vi "OFDM_SuperpositionedBitDetectV3.vi"(5 "Alpha":dbl, 6 "Input symbolsLP":cdb[](array[numeric]) format="%.2f", 7 "Input symbolsHP":cdb[](array[numeric]) format="%.2f", 8 "error in (no error)":errorcluster, 9 "Modulation type LP":enum16{"QPSK(4QAM)", "64QAM", "16QAM", "BPSK"}(ring), 10 "Modulation type":enum16{"QPSK(4QAM)", "64QAM", "16QAM", "BPSK"}(ring), 11 "Input symbols":cdb[](array[numeric]) format="%.2f") -> (0 "error out":errorcluster, 1 "OutputbitsHP":i8[](array[numeric]) caption="Output bits", 2 "SNR dB HP":dbl, 3 "OutputbitsLP":i8[](array[numeric]) caption="Output bits", 4 "SNR dB LP":dbl)   [LabVIEW 2022 SP3]
uses:
  <vilib>/addons/Modulation/Digital/General/MT Map QAM Symbols to Bits.vi
  <vilib>/addons/Modulation/Digital/General/MT Map Bits to QAM Symbols.vi
  <vilib>/addons/Modulation/Digital/General/MT Map PSK Symbols to Bits.vi
  <vilib>/addons/Modulation/Digital/General/MT Map Bits to PSK Symbols.vi
  <vilib>/addons/Modulation/niDMT.lvlib
panel:
  out "x-y":cdb[](array[numeric])
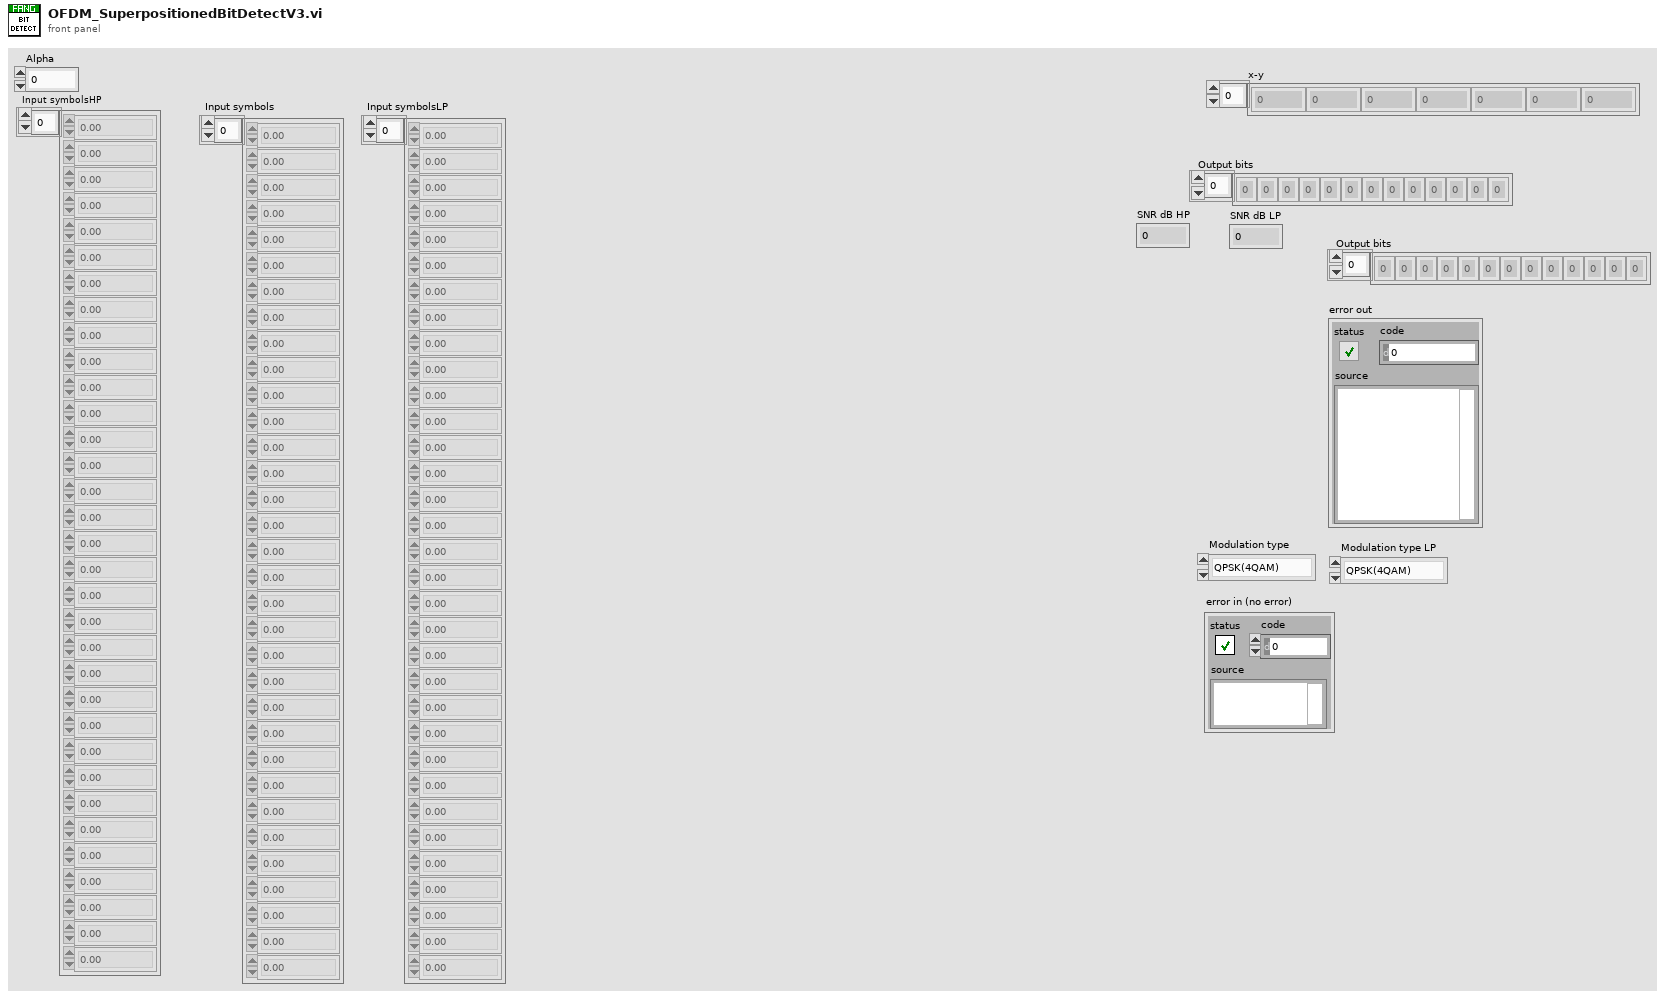
[diagram p1: front panel]
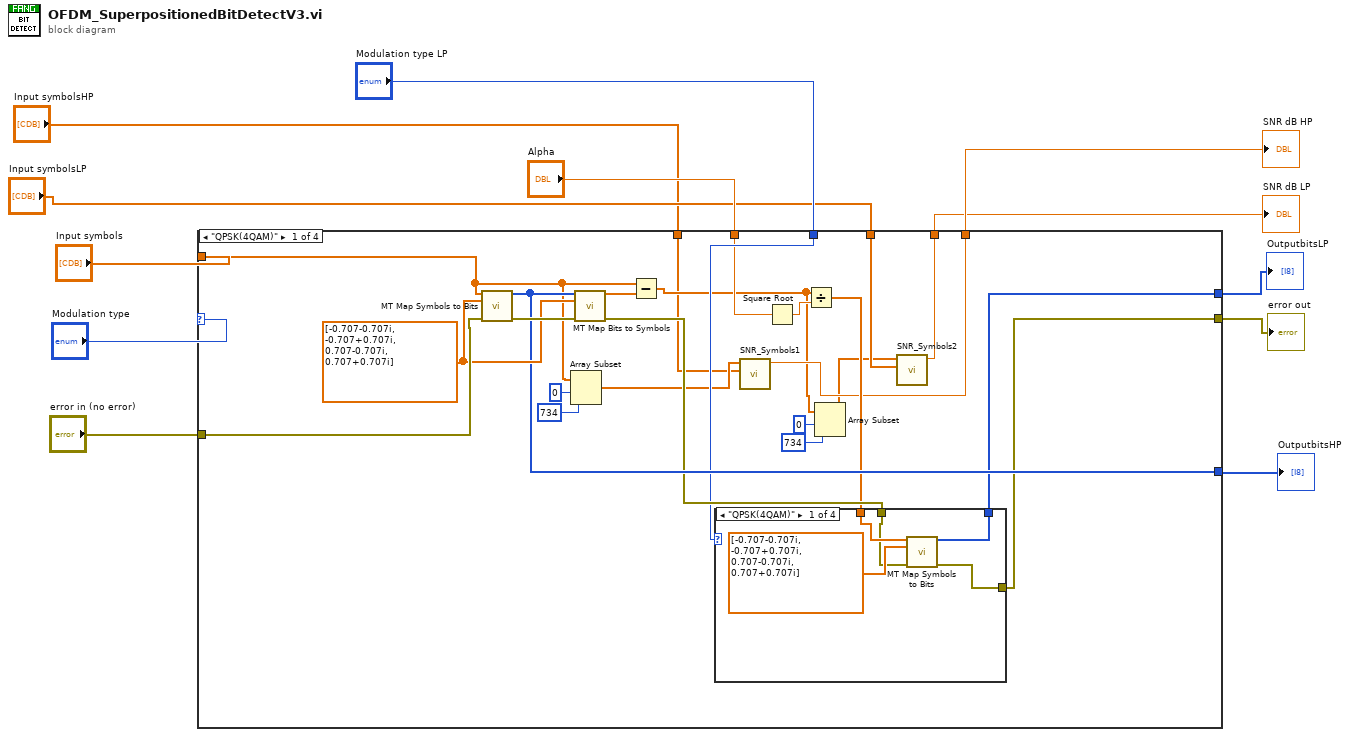
[diagram p0: block diagram]
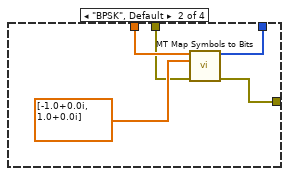
[diagram p2: hidden frame]
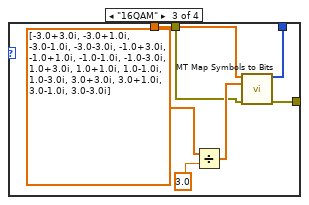
[diagram p3: hidden frame]
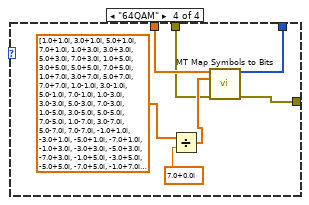
[diagram p4: hidden frame]
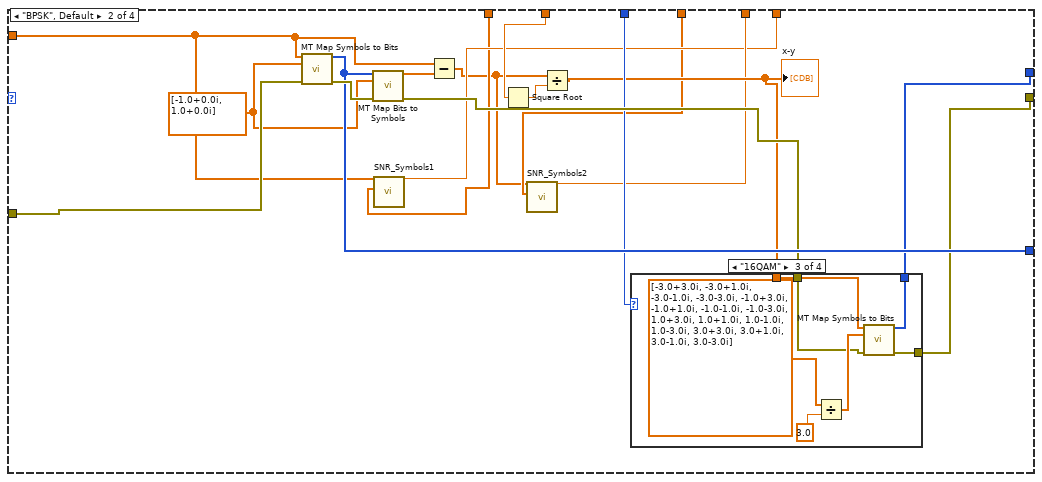
[diagram p5: hidden frame]
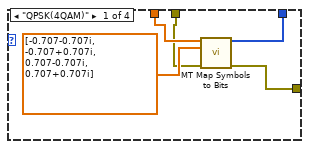
[diagram p6: hidden frame]
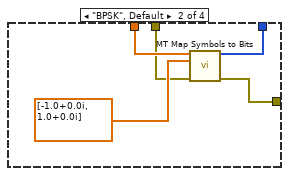
[diagram p7: hidden frame]
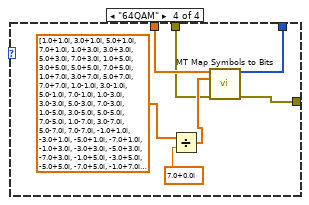
[diagram p8: hidden frame]
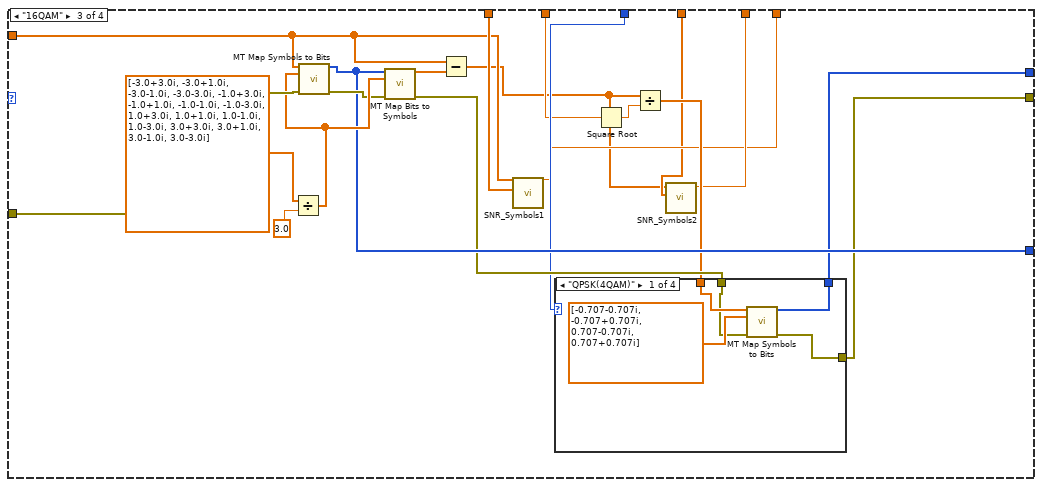
[diagram p9: hidden frame]
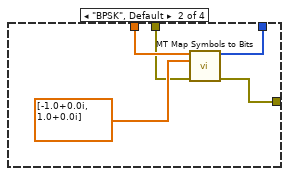
[diagram p10: hidden frame]
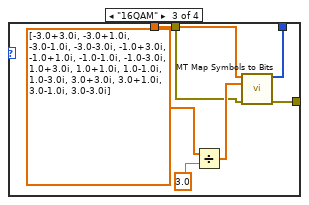
[diagram p11: hidden frame]
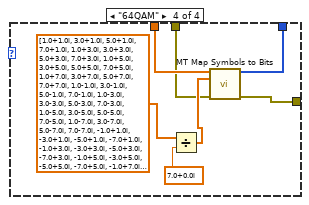
[diagram p12: hidden frame]
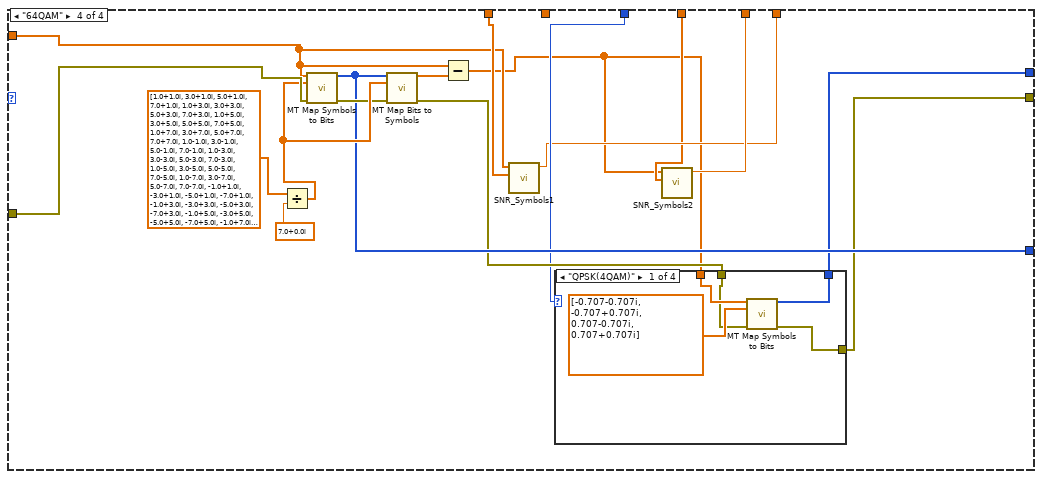
[diagram p13: hidden frame]
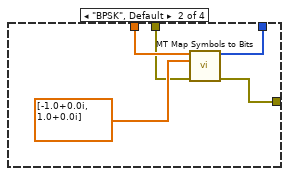
[diagram p14: hidden frame]
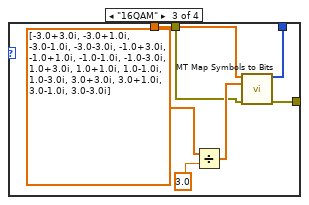
[diagram p15: hidden frame]
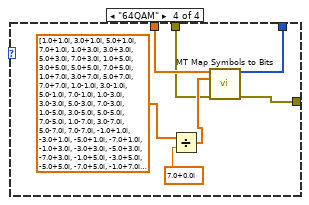
[diagram p16: hidden frame]
diagram:
  n1 = case shown="\"QPSK(4QAM)\"" "Modulation type" {
    tunnel: "Input symbols" -> [w14 w62 w104 w148]
    tunnel: "error in (no error)" -> [w36 w78 w122 w161]
    tunnel: [w30 w73 w113 w154] -> w9
    tunnel: [w31 w72 w114 w155] -> w8
    tunnel: [w33 w75 w116 w157] -> w7
    tunnel: "Modulation type LP" -> [w29 w70 w112 w153]
    tunnel: "Alpha" -> [w26 w67 w109 _]
    tunnel: "Input symbolsHP" -> [w15 w64 w106 w150]
    tunnel: "Input symbolsLP" -> [w25 w63 w105 w149]
    tunnel: [w24 w65 w107 w151] -> w3
    tunnel: [w23 w66 w108 w152] -> w2
    frame "QPSK(4QAM)" {
      w34 = cdb[] [-0.707-0.707i, -0.707+0.707i, 0.707-0.707i, 0.707+0.707i] ("symbol map")
      n2 = call-poly <vilib>:"MT Map Symbols to Bits.vi"("symbols"=w14, "symbol map"=w34, "error in (no error)"=w36) -> ("output bit stream"=w33:i8[], "error out"=w35:errorcluster)  [unwired: 11 in]
      n3 = Array Subset(array=w14, index=0, length=734) -> (w22:cdb[])
      n4 = call-poly <vilib>:"MT Map Bits to Symbols.vi"("input bit stream"=w33, "symbol map"=w34, "error in (no error)"=w35) -> ("symbols"=w13:cdb[], "error out"=w32:errorcluster)  [unwired: 11 in]
      n5 = Subtract(x=w14, y=w13) -> (x-y=w16:cdb[])
      n6 = call "SNR_Symbols1.vi"("Ideal Symbols"=w15, "Received symbols"=w22) -> ("SNR dB"=w24:dbl)  [unwired: 9 in]
      n7 = Square Root(x=w26) -> (sqrt(x)=w28:dbl)
      n8 = Divide(x=w16, y=w28) -> (x/y=w27:cdb[])
      n9 = case shown="\"QPSK(4QAM)\"" w29 {
        tunnel: w27 -> [w40 w45 w50 w57]
        tunnel: [w38 w44 w49 w55] -> w30
        tunnel: [w37 w42 w48 w54] -> w31
        tunnel: w32 -> [w39 w43 w47 w56]
        frame "QPSK(4QAM)" {
          n10 = call-poly <vilib>:"MT Map Symbols to Bits.vi"("symbols"=w40, "symbol map"=cdb[] [-0.707-0.707i, -0.707+0.707i, 0.707-0.707i, 0.707+0.707i], "error in (no error)"=w39) -> ("output bit stream"=w38:i8[], "error out"=w37:errorcluster)  [unwired: 11 in]
        }
        frame "BPSK", Default {
          n11 = call-poly <vilib>:"MT Map Symbols to Bits.vi"("symbols"=w45, "symbol map"=cdb[] [-1.0+0.0i, 1.0+0.0i], "error in (no error)"=w43) -> ("output bit stream"=w44:i8[], "error out"=w42:errorcluster)  [unwired: 11 in]
        }
        frame "16QAM" {
          n12 = Divide(x=cdb[] [-3.0+3.0i, -3.0+1.0i, -3.0-1.0i, -3.0-3.0i, -1.0+3.0i, -1.0+1.0i, -1.0-1.0i, -1.0-3.0i, 1.0+3.0i, 1.0+1.0i, 1.0-1.0i, 1.0-3.0i, 3.0+3.0i, 3.0+1.0i, 3.0-1.0i, 3.0-3.0i] ("symbol map"), y=3.0) -> (x/y=w51:cdb[])
          n13 = call-poly <vilib>:"MT Map Symbols to Bits.vi"("symbols"=w50, "symbol map"=w51, "error in (no error)"=w47) -> ("output bit stream"=w49:i8[], "error out"=w48:errorcluster)  [unwired: 11 in]
        }
        frame "64QAM" {
          n14 = Divide(x=cdb[] [1.0+1.0i, 3.0+1.0i, 5.0+1.0i, 7.0+1.0i, 1.0+3.0i, 3.0+3.0i, 5.0+3.0i, 7.0+3.0i, 1.0+5.0i, 3.0+5.0i, 5.0+5.0i, 7.0+5.0i, 1.0+7.0i, 3.0+7.0i, 5.0+7.0i, 7.0+7.0i, 1.0-1.0i, 3.0-1.0i, 5.0-1.0i, 7.0-1.0i, 1.0-3.0i, 3.0-3.0i, 5.0-3.0i, 7.0-3.0i, 1.0-5.0i, 3.0-5.0i, 5.0-5.0i, 7.0-5.0i, 1.0-7.0i, 3.0-7.0i, 5.0-7.0i, 7.0-7.0i, -1.0+1.0i, -3.0+1.0i, -5.0+1.0i, -7.0+1.0i, -1.0+3.0i, -3.0+3.0i, -5.0+3.0i, -7.0+3.0i, -1.0+5.0i, -3.0+5.0i, -5.0+5.0i, -7.0+5.0i, -1.0+7.0i, -3.0+7.0i, -5.0+7.0i, -7.0+7.0i, -1.0-1.0i, -3.0-1.0i, -5.0-1.0i, -7.0-1.0i, -1.0-3.0i, -3.0-3.0i, -5.0-3.0i, -7.0-3.0i, -1.0-5.0i, -3.0-5.0i, -5.0-5.0i, -7.0-5.0i, -1.0-7.0i, -3.0-7.0i, -5.0-7.0i, -7.0-7.0i] ("appended array"), y=cdb 7.0+0.0i) -> (x/y=w58:cdb[])
          n15 = call-poly <vilib>:"MT Map Symbols to Bits.vi"("symbols"=w57, "symbol map"=w58, "error in (no error)"=w56) -> ("output bit stream"=w55:i8[], "error out"=w54:errorcluster)  [unwired: 11 in]
        }
      }
      n16 = Array Subset(array=w16, index=0, length=734) -> (w17:cdb[])
      n17 = call "SNR_Symbols2.vi"("Ideal Symbols"=w25, "Received symbols"=w17) -> ("SNR dB"=w23:dbl)  [unwired: 9 in]
    }
    frame "BPSK", Default {
      w74 = cdb[] [-1.0+0.0i, 1.0+0.0i] ("symbol map")
      n18 = call-poly <vilib>:"MT Map Symbols to Bits.vi"("symbols"=w62, "symbol map"=w74, "error in (no error)"=w78) -> ("output bit stream"=w75:i8[], "error out"=w77:errorcluster)  [unwired: 11 in]
      n19 = call-poly <vilib>:"MT Map Bits to Symbols.vi"("input bit stream"=w75, "symbol map"=w74, "error in (no error)"=w77) -> ("symbols"=w76:cdb[], "error out"=w71:errorcluster)  [unwired: 11 in]
      n20 = call "SNR_Symbols1.vi"("Ideal Symbols"=w64, "Received symbols"=w62) -> ("SNR dB"=w65:dbl)  [unwired: 9 in]
      n21 = Subtract(x=w62, y=w76) -> (x-y=w61:cdb[])
      n22 = Square Root(x=w67) -> (sqrt(x)=w68:dbl)
      n23 = call "SNR_Symbols2.vi"("Ideal Symbols"=w63, "Received symbols"=w61) -> ("SNR dB"=w66:dbl)  [unwired: 9 in]
      n24 = Divide(x=w61, y=w68) -> (x/y=w69:cdb[])
      "x-y" <- w69
      n25 = case shown="\"16QAM\"" w70 {
        tunnel: w69 -> [w82 w87 w92 w99]
        tunnel: [w80 w86 w91 w97] -> w73
        tunnel: [w79 w84 w90 w96] -> w72
        tunnel: w71 -> [w81 w85 w89 w98]
        frame "QPSK(4QAM)" {
          n26 = call-poly <vilib>:"MT Map Symbols to Bits.vi"("symbols"=w82, "symbol map"=cdb[] [-0.707-0.707i, -0.707+0.707i, 0.707-0.707i, 0.707+0.707i], "error in (no error)"=w81) -> ("output bit stream"=w80:i8[], "error out"=w79:errorcluster)  [unwired: 11 in]
        }
        frame "BPSK", Default {
          n27 = call-poly <vilib>:"MT Map Symbols to Bits.vi"("symbols"=w87, "symbol map"=cdb[] [-1.0+0.0i, 1.0+0.0i], "error in (no error)"=w85) -> ("output bit stream"=w86:i8[], "error out"=w84:errorcluster)  [unwired: 11 in]
        }
        frame "16QAM" {
          n28 = Divide(x=cdb[] [-3.0+3.0i, -3.0+1.0i, -3.0-1.0i, -3.0-3.0i, -1.0+3.0i, -1.0+1.0i, -1.0-1.0i, -1.0-3.0i, 1.0+3.0i, 1.0+1.0i, 1.0-1.0i, 1.0-3.0i, 3.0+3.0i, 3.0+1.0i, 3.0-1.0i, 3.0-3.0i] ("symbol map"), y=3.0) -> (x/y=w93:cdb[])
          n29 = call-poly <vilib>:"MT Map Symbols to Bits.vi"("symbols"=w92, "symbol map"=w93, "error in (no error)"=w89) -> ("output bit stream"=w91:i8[], "error out"=w90:errorcluster)  [unwired: 11 in]
        }
        frame "64QAM" {
          n30 = Divide(x=cdb[] [1.0+1.0i, 3.0+1.0i, 5.0+1.0i, 7.0+1.0i, 1.0+3.0i, 3.0+3.0i, 5.0+3.0i, 7.0+3.0i, 1.0+5.0i, 3.0+5.0i, 5.0+5.0i, 7.0+5.0i, 1.0+7.0i, 3.0+7.0i, 5.0+7.0i, 7.0+7.0i, 1.0-1.0i, 3.0-1.0i, 5.0-1.0i, 7.0-1.0i, 1.0-3.0i, 3.0-3.0i, 5.0-3.0i, 7.0-3.0i, 1.0-5.0i, 3.0-5.0i, 5.0-5.0i, 7.0-5.0i, 1.0-7.0i, 3.0-7.0i, 5.0-7.0i, 7.0-7.0i, -1.0+1.0i, -3.0+1.0i, -5.0+1.0i, -7.0+1.0i, -1.0+3.0i, -3.0+3.0i, -5.0+3.0i, -7.0+3.0i, -1.0+5.0i, -3.0+5.0i, -5.0+5.0i, -7.0+5.0i, -1.0+7.0i, -3.0+7.0i, -5.0+7.0i, -7.0+7.0i, -1.0-1.0i, -3.0-1.0i, -5.0-1.0i, -7.0-1.0i, -1.0-3.0i, -3.0-3.0i, -5.0-3.0i, -7.0-3.0i, -1.0-5.0i, -3.0-5.0i, -5.0-5.0i, -7.0-5.0i, -1.0-7.0i, -3.0-7.0i, -5.0-7.0i, -7.0-7.0i] ("appended array"), y=cdb 7.0+0.0i) -> (x/y=w100:cdb[])
          n31 = call-poly <vilib>:"MT Map Symbols to Bits.vi"("symbols"=w99, "symbol map"=w100, "error in (no error)"=w98) -> ("output bit stream"=w97:i8[], "error out"=w96:errorcluster)  [unwired: 11 in]
        }
      }
    }
    frame "16QAM" {
      n32 = Divide(x=cdb[] [-3.0+3.0i, -3.0+1.0i, -3.0-1.0i, -3.0-3.0i, -1.0+3.0i, -1.0+1.0i, -1.0-1.0i, -1.0-3.0i, 1.0+3.0i, 1.0+1.0i, 1.0-1.0i, 1.0-3.0i, 3.0+3.0i, 3.0+1.0i, 3.0-1.0i, 3.0-3.0i] ("symbol map"), y=3.0) -> (x/y=w119:cdb[])
      n33 = call-poly <vilib>:"MT Map Symbols to Bits.vi"("symbols"=w104, "symbol map"=w119, "error in (no error)"=w122) -> ("output bit stream"=w116:i8[], "error out"=w117:errorcluster)  [unwired: 11 in]
      n34 = call-poly <vilib>:"MT Map Bits to Symbols.vi"("input bit stream"=w116, "symbol map"=w119, "error in (no error)"=w117) -> ("symbols"=w118:cdb[], "error out"=w115:errorcluster)  [unwired: 11 in]
      n35 = Subtract(x=w104, y=w118) -> (x-y=w103:cdb[])
      n36 = call "SNR_Symbols1.vi"("Ideal Symbols"=w106, "Received symbols"=w104) -> ("SNR dB"=w107:dbl)  [unwired: 9 in]
      n37 = Square Root(x=w109) -> (sqrt(x)=w111:dbl)
      n38 = Divide(x=w103, y=w111) -> (x/y=w110:cdb[])
      n39 = case shown="\"QPSK(4QAM)\"" w112 {
        tunnel: w110 -> [w126 w131 w136 w143]
        tunnel: [w124 w130 w135 w141] -> w113
        tunnel: [w123 w128 w134 w140] -> w114
        tunnel: w115 -> [w125 w129 w133 w142]
        frame "QPSK(4QAM)" {
          n40 = call-poly <vilib>:"MT Map Symbols to Bits.vi"("symbols"=w126, "symbol map"=cdb[] [-0.707-0.707i, -0.707+0.707i, 0.707-0.707i, 0.707+0.707i], "error in (no error)"=w125) -> ("output bit stream"=w124:i8[], "error out"=w123:errorcluster)  [unwired: 11 in]
        }
        frame "BPSK", Default {
          n41 = call-poly <vilib>:"MT Map Symbols to Bits.vi"("symbols"=w131, "symbol map"=cdb[] [-1.0+0.0i, 1.0+0.0i], "error in (no error)"=w129) -> ("output bit stream"=w130:i8[], "error out"=w128:errorcluster)  [unwired: 11 in]
        }
        frame "16QAM" {
          n42 = Divide(x=cdb[] [-3.0+3.0i, -3.0+1.0i, -3.0-1.0i, -3.0-3.0i, -1.0+3.0i, -1.0+1.0i, -1.0-1.0i, -1.0-3.0i, 1.0+3.0i, 1.0+1.0i, 1.0-1.0i, 1.0-3.0i, 3.0+3.0i, 3.0+1.0i, 3.0-1.0i, 3.0-3.0i] ("symbol map"), y=3.0) -> (x/y=w137:cdb[])
          n43 = call-poly <vilib>:"MT Map Symbols to Bits.vi"("symbols"=w136, "symbol map"=w137, "error in (no error)"=w133) -> ("output bit stream"=w135:i8[], "error out"=w134:errorcluster)  [unwired: 11 in]
        }
        frame "64QAM" {
          n44 = Divide(x=cdb[] [1.0+1.0i, 3.0+1.0i, 5.0+1.0i, 7.0+1.0i, 1.0+3.0i, 3.0+3.0i, 5.0+3.0i, 7.0+3.0i, 1.0+5.0i, 3.0+5.0i, 5.0+5.0i, 7.0+5.0i, 1.0+7.0i, 3.0+7.0i, 5.0+7.0i, 7.0+7.0i, 1.0-1.0i, 3.0-1.0i, 5.0-1.0i, 7.0-1.0i, 1.0-3.0i, 3.0-3.0i, 5.0-3.0i, 7.0-3.0i, 1.0-5.0i, 3.0-5.0i, 5.0-5.0i, 7.0-5.0i, 1.0-7.0i, 3.0-7.0i, 5.0-7.0i, 7.0-7.0i, -1.0+1.0i, -3.0+1.0i, -5.0+1.0i, -7.0+1.0i, -1.0+3.0i, -3.0+3.0i, -5.0+3.0i, -7.0+3.0i, -1.0+5.0i, -3.0+5.0i, -5.0+5.0i, -7.0+5.0i, -1.0+7.0i, -3.0+7.0i, -5.0+7.0i, -7.0+7.0i, -1.0-1.0i, -3.0-1.0i, -5.0-1.0i, -7.0-1.0i, -1.0-3.0i, -3.0-3.0i, -5.0-3.0i, -7.0-3.0i, -1.0-5.0i, -3.0-5.0i, -5.0-5.0i, -7.0-5.0i, -1.0-7.0i, -3.0-7.0i, -5.0-7.0i, -7.0-7.0i] ("appended array"), y=cdb 7.0+0.0i) -> (x/y=w144:cdb[])
          n45 = call-poly <vilib>:"MT Map Symbols to Bits.vi"("symbols"=w143, "symbol map"=w144, "error in (no error)"=w142) -> ("output bit stream"=w141:i8[], "error out"=w140:errorcluster)  [unwired: 11 in]
        }
      }
      n46 = call "SNR_Symbols2.vi"("Ideal Symbols"=w105, "Received symbols"=w103) -> ("SNR dB"=w108:dbl)  [unwired: 9 in]
    }
    frame "64QAM" {
      n47 = Divide(x=cdb[] [1.0+1.0i, 3.0+1.0i, 5.0+1.0i, 7.0+1.0i, 1.0+3.0i, 3.0+3.0i, 5.0+3.0i, 7.0+3.0i, 1.0+5.0i, 3.0+5.0i, 5.0+5.0i, 7.0+5.0i, 1.0+7.0i, 3.0+7.0i, 5.0+7.0i, 7.0+7.0i, 1.0-1.0i, 3.0-1.0i, 5.0-1.0i, 7.0-1.0i, 1.0-3.0i, 3.0-3.0i, 5.0-3.0i, 7.0-3.0i, 1.0-5.0i, 3.0-5.0i, 5.0-5.0i, 7.0-5.0i, 1.0-7.0i, 3.0-7.0i, 5.0-7.0i, 7.0-7.0i, -1.0+1.0i, -3.0+1.0i, -5.0+1.0i, -7.0+1.0i, -1.0+3.0i, -3.0+3.0i, -5.0+3.0i, -7.0+3.0i, -1.0+5.0i, -3.0+5.0i, -5.0+5.0i, -7.0+5.0i, -1.0+7.0i, -3.0+7.0i, -5.0+7.0i, -7.0+7.0i, -1.0-1.0i, -3.0-1.0i, -5.0-1.0i, -7.0-1.0i, -1.0-3.0i, -3.0-3.0i, -5.0-3.0i, -7.0-3.0i, -1.0-5.0i, -3.0-5.0i, -5.0-5.0i, -7.0-5.0i, -1.0-7.0i, -3.0-7.0i, -5.0-7.0i, -7.0-7.0i] ("appended array"), y=cdb 7.0+0.0i) -> (x/y=w160:cdb[])
      n48 = call-poly <vilib>:"MT Map Symbols to Bits.vi"("symbols"=w148, "symbol map"=w160, "error in (no error)"=w161) -> ("output bit stream"=w157:i8[], "error out"=w158:errorcluster)  [unwired: 11 in]
      n49 = call-poly <vilib>:"MT Map Bits to Symbols.vi"("input bit stream"=w157, "symbol map"=w160, "error in (no error)"=w158) -> ("symbols"=w159:cdb[], "error out"=w156:errorcluster)  [unwired: 11 in]
      n50 = Subtract(x=w148, y=w159) -> (x-y=w147:cdb[])
      n51 = call "SNR_Symbols1.vi"("Ideal Symbols"=w150, "Received symbols"=w148) -> ("SNR dB"=w151:dbl)  [unwired: 9 in]
      n52 = case shown="\"QPSK(4QAM)\"" w153 {
        tunnel: w147 -> [w167 w172 w177 w184]
        tunnel: [w165 w171 w176 w182] -> w154
        tunnel: [w164 w169 w175 w181] -> w155
        tunnel: w156 -> [w166 w170 w174 w183]
        frame "QPSK(4QAM)" {
          n53 = call-poly <vilib>:"MT Map Symbols to Bits.vi"("symbols"=w167, "symbol map"=cdb[] [-0.707-0.707i, -0.707+0.707i, 0.707-0.707i, 0.707+0.707i], "error in (no error)"=w166) -> ("output bit stream"=w165:i8[], "error out"=w164:errorcluster)  [unwired: 11 in]
        }
        frame "BPSK", Default {
          n54 = call-poly <vilib>:"MT Map Symbols to Bits.vi"("symbols"=w172, "symbol map"=cdb[] [-1.0+0.0i, 1.0+0.0i], "error in (no error)"=w170) -> ("output bit stream"=w171:i8[], "error out"=w169:errorcluster)  [unwired: 11 in]
        }
        frame "16QAM" {
          n55 = Divide(x=cdb[] [-3.0+3.0i, -3.0+1.0i, -3.0-1.0i, -3.0-3.0i, -1.0+3.0i, -1.0+1.0i, -1.0-1.0i, -1.0-3.0i, 1.0+3.0i, 1.0+1.0i, 1.0-1.0i, 1.0-3.0i, 3.0+3.0i, 3.0+1.0i, 3.0-1.0i, 3.0-3.0i] ("symbol map"), y=3.0) -> (x/y=w178:cdb[])
          n56 = call-poly <vilib>:"MT Map Symbols to Bits.vi"("symbols"=w177, "symbol map"=w178, "error in (no error)"=w174) -> ("output bit stream"=w176:i8[], "error out"=w175:errorcluster)  [unwired: 11 in]
        }
        frame "64QAM" {
          n57 = Divide(x=cdb[] [1.0+1.0i, 3.0+1.0i, 5.0+1.0i, 7.0+1.0i, 1.0+3.0i, 3.0+3.0i, 5.0+3.0i, 7.0+3.0i, 1.0+5.0i, 3.0+5.0i, 5.0+5.0i, 7.0+5.0i, 1.0+7.0i, 3.0+7.0i, 5.0+7.0i, 7.0+7.0i, 1.0-1.0i, 3.0-1.0i, 5.0-1.0i, 7.0-1.0i, 1.0-3.0i, 3.0-3.0i, 5.0-3.0i, 7.0-3.0i, 1.0-5.0i, 3.0-5.0i, 5.0-5.0i, 7.0-5.0i, 1.0-7.0i, 3.0-7.0i, 5.0-7.0i, 7.0-7.0i, -1.0+1.0i, -3.0+1.0i, -5.0+1.0i, -7.0+1.0i, -1.0+3.0i, -3.0+3.0i, -5.0+3.0i, -7.0+3.0i, -1.0+5.0i, -3.0+5.0i, -5.0+5.0i, -7.0+5.0i, -1.0+7.0i, -3.0+7.0i, -5.0+7.0i, -7.0+7.0i, -1.0-1.0i, -3.0-1.0i, -5.0-1.0i, -7.0-1.0i, -1.0-3.0i, -3.0-3.0i, -5.0-3.0i, -7.0-3.0i, -1.0-5.0i, -3.0-5.0i, -5.0-5.0i, -7.0-5.0i, -1.0-7.0i, -3.0-7.0i, -5.0-7.0i, -7.0-7.0i] ("appended array"), y=cdb 7.0+0.0i) -> (x/y=w185:cdb[])
          n58 = call-poly <vilib>:"MT Map Symbols to Bits.vi"("symbols"=w184, "symbol map"=w185, "error in (no error)"=w183) -> ("output bit stream"=w182:i8[], "error out"=w181:errorcluster)  [unwired: 11 in]
        }
      }
      n59 = call "SNR_Symbols2.vi"("Ideal Symbols"=w149, "Received symbols"=w147) -> ("SNR dB"=w152:dbl)  [unwired: 9 in]
    }
  }
  "OutputbitsLP" <- w9
  "error out" <- w8
  "OutputbitsHP" <- w7
  "SNR dB HP" <- w3
  "SNR dB LP" <- w2
